vi "closeVisaMaybe.vi"(8 "VISA resource name in":refnum<visa-resource-name>, 9 "error in":errorcluster, 11 "VISA connected?":bool) -> (1 "error out":errorcluster)   [LabVIEW 2025]
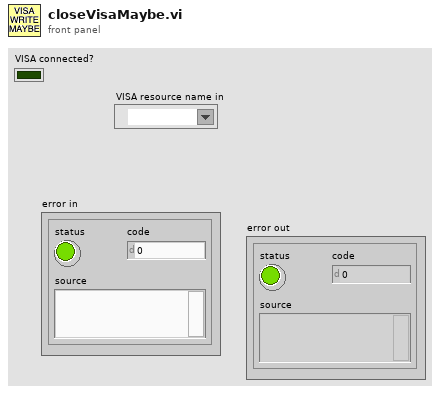
[diagram p1: front panel]
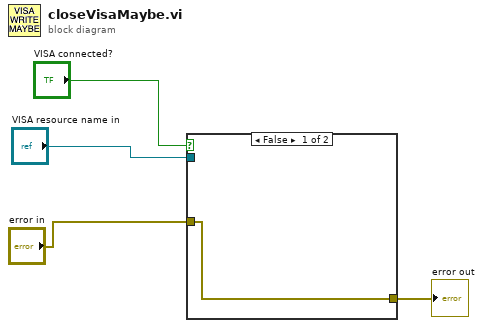
[diagram p0: block diagram]
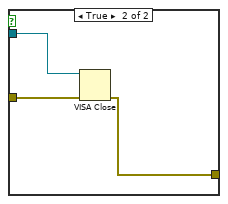
[diagram p2: hidden frame]
diagram:
  n1 = case shown="False" "VISA connected?" {
    tunnel: "VISA resource name in" -> [_ w8]
    tunnel: "error in" -> [w5 w7]
    tunnel: [w5 w6] -> w1
    frame False {
    }
    frame True {
      n2 = VISA Close(VISA resource name=w8, error in (no error)=w7) -> (error out=w6:errorcluster)
    }
  }
  "error out" <- w1
